vi "Regex XNode Call.vi"(0 "input string":string, 5 "regular expression":string, 7 "ignore case?":bool, 11 "error in":errorcluster) -> (4 "before match":string, 6 "whole match":string, 8 "after match":string, 10 "offset past match":i32, 15 "error out":errorcluster)   [LabVIEW 2026]
doc: "Finds the first match of a regular expression with LabVIEW's Match Regular Expression XNode and returns the text before, in and after it."
uses:
  <vilib>/regexp/Match Regular Expression.xnode
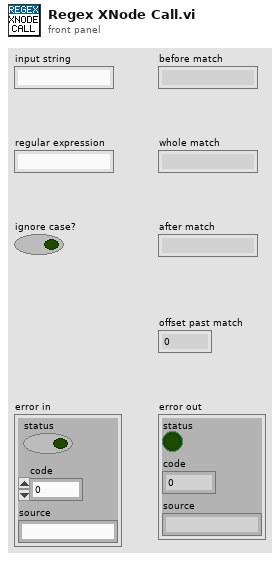
[diagram p1: front panel]
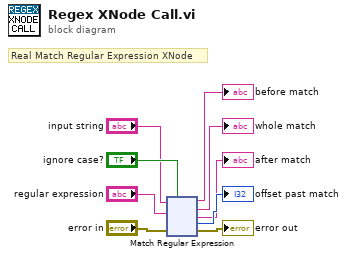
[diagram p0: block diagram]
diagram:
  # "Real Match Regular Expression XNode"
  n1 = xnode "Match Regular Expression"("input string"="input string", "regular expression"="regular expression", "error in"="error in", "ignore case? (F)"="ignore case?") -> ("before match"=→"before match":string, "whole match"=→"whole match":string, "after match"=→"after match":string, "offset past match"=→"offset past match":i32, "error out"=→"error out":errorcluster)  [unwired: 2 in]
